vi "VIH HelpGen - FILE - Get Type of Invalid.vi"(8 "error in":errorcluster, 10 "File Type":T1, 11 "File Path":path) -> (0 "error out":errorcluster, 1 "Not found":bool, 2 "File Type out":T1, 3 "File Path out":path)   [LabVIEW 2014]
doc: "::: VI Helpeks :::\nCopyright (c) 2000-2026 Konstantin Shifershteyn. All rights reserved."
uses:
  _VIH HelpGen - Palette.llb/VIH HelpGen Typedef - Palette - Item Type Enum.ctl
panel:
  # "VI Helpeks\nCopyright (c) 2012-2026 Konstantin Shifershteyn"
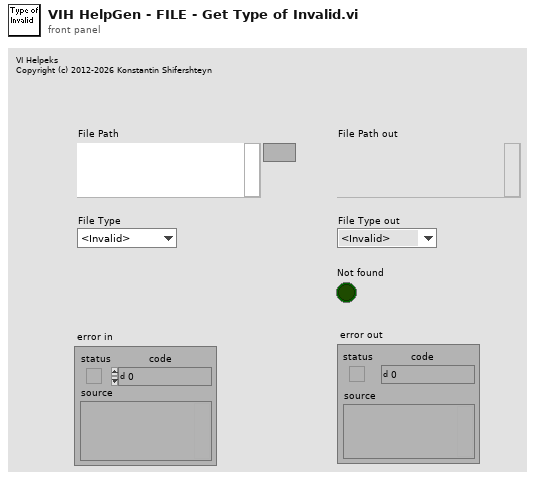
[diagram p1: front panel]
types:
  T1 = typedef "VIH HelpGen Typedef - Palette - Item Type Enum.ctl" = enum32{"<Invalid>", "<unknown>", "VI", "Menu", "LV Func", "Express VI", "Poly VI", "CTL", "HTML"}
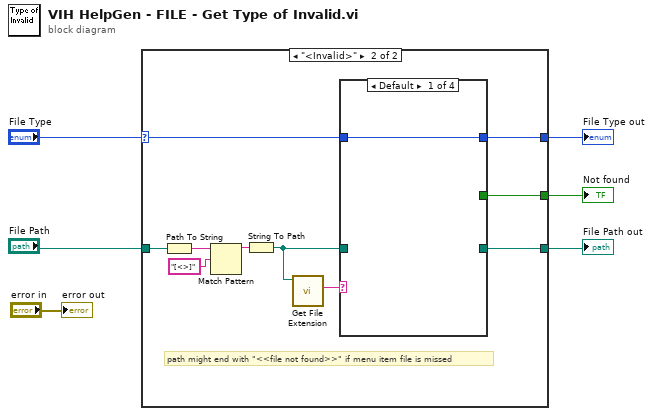
[diagram p0: block diagram]
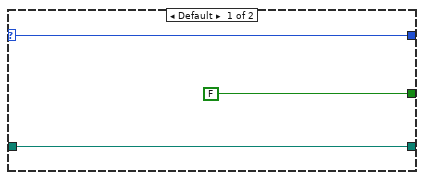
[diagram p2: hidden frame]
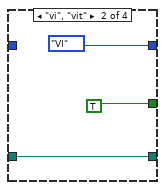
[diagram p3: hidden frame]
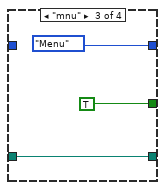
[diagram p4: hidden frame]
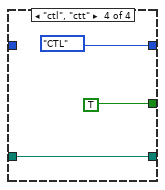
[diagram p5: hidden frame]
diagram:
  n1 = case shown="\"<Invalid>\"" "File Type" {
    selector: "File Type" -> [w9 w11]
    tunnel: [w8 w13] -> w4
    tunnel: "File Path" -> [w8 w17]
    tunnel: [w9 w12] -> w2
    tunnel: [FALSE w10] -> w1
    frame Default {
    }
    frame "<Invalid>" {
      # "path might end with \"<<file not found>>\" if menu item file is missed"
      n2 = Path To String(path=w17) -> (string=w19:string)
      n3 = Match Pattern(string=w19, regular expression="[<>]") -> (before substring=w16:string)  [unwired: 1 in, 3 out]
      n4 = String To Path(string=w16) -> (path=w14:path)
      n5 = call <vilib>:"Get File Extension.vi"("file"=w14) -> ("lowercase file extension"=w15:string)  [unwired: 7 in, 3 out]
      n6 = case shown="Default" w15 {
        tunnel: w14 -> [_ w23 w26 w29]
        tunnel: [_ w23 w26 w29] -> w13
        tunnel: [w20 VIH_HelpGen_Typedef_-_Palette_-_Item_Type_Enum."VI" ("File Type") VIH_HelpGen_Typedef_-_Palette_-_Item_Type_Enum."Menu" ("File Type") VIH_HelpGen_Typedef_-_Palette_-_Item_Type_Enum."CTL" ("File Type")] -> w12
        tunnel: w11 -> [w20 _ _ _]
        tunnel: [_ TRUE TRUE TRUE] -> w10
        frame Default {
        }
        frame "vi", "vit" {
        }
        frame "mnu" {
        }
        frame "ctl", "ctt" {
        }
      }
    }
  }
  "File Path out" <- w4
  "File Type out" <- w2
  "Not found" <- w1
  "error out" <- "error in"
